vi "Get XML.vi"(8 "error in (no error)":errorcluster, 11 "ToastFromXML in":refnum<class "ToastFromXML.lvclass">) -> (0 "error out":errorcluster, 2 "GetContent":string, 3 "ToastFromXML out":refnum<class "ToastFromXML.lvclass">)   [LabVIEW 2026, in "ToastNotification.lvlib" / "ToastFromXML.lvclass"]
doc: "Serialize the retained XML Document into the GetContent LabVIEW string. Skipped on incoming error. Returns the same ToastFromXML without displaying or closing it; the temporary boxed string is released. Serialization may normalize the original XML formatting. The caller retains ownership of Close."
uses:
  ToastFromXML.lvclass
  ToastFromXML.lvclass/ToastFromXML.ctl
  Read XML Document.vi
  Reflection DotNet/Reflection DotNet.lvlib
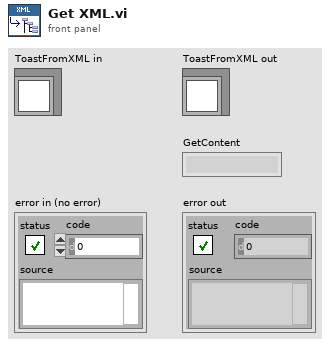
[diagram p1: front panel]
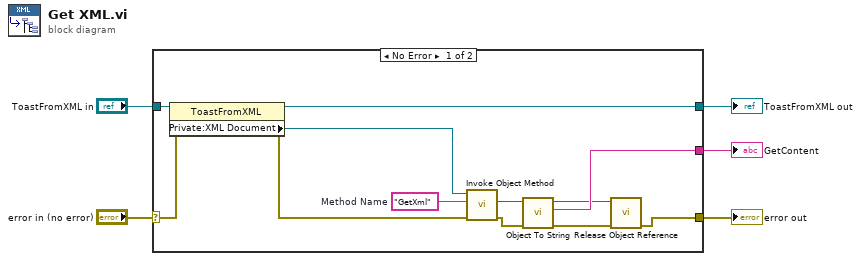
[diagram p0: block diagram]
diagram:
  n1 = case shown="No Error" "error in (no error)" {
    selector: "error in (no error)" -> [w15 w18]
    tunnel: [w16 w19] -> w4
    tunnel: "ToastFromXML in" -> [w17 w19]
    tunnel: [w6 w18] -> w2
    tunnel: [w9 _] -> w1
    frame No Error {
      w12 = "GetXml"  # Method Name
      n2 = property class="ToastFromXML"(reference=w17, error in=w15) -> (reference out=w16:refnum<class "ToastFromXML.lvclass">, error out=w14:errorcluster, "Private:XML Document"=w13:refnum<k24>)
      n3 = call "Invoke Object Method.vi"("error in"=w14, "Method Name"=w12, "Object in"=w13) -> ("error out"=w11:errorcluster, "Return Value"=w10:refnum<k24>)  [unwired: 6 in, 1 out]
      n4 = call "Object To String.vi"("error in (no error)"=w11, "Object in"=w10) -> ("error out"=w7:errorcluster, "Text"=w9:string, "Object out"=w8:refnum<k24>)  [unwired: 7 in]
      n5 = call "Release Object Reference.vi"("error in"=w7, "object"=w8) -> ("error out"=w6:errorcluster)  [unwired: 9 in]
    }
    frame Error {
    }
  }
  "error out" <- w2
  "ToastFromXML out" <- w4
  "GetContent" <- w1
